vi "Read ApplicationRef.vi"(8 "error in (no error)":errorcluster, 11 "Test Runner in":refnum<class "Test Runner.lvclass">) -> (0 "error out":errorcluster, 2 "Application":refnum<vi>, 3 "Test Runner out":refnum<class "Test Runner.lvclass">)   [LabVIEW 2020, in "Caraya.lvlib" / "Test Runner.lvclass"]
uses:
  Test Runner.lvclass
  Test Runner.lvclass/Test Runner.ctl
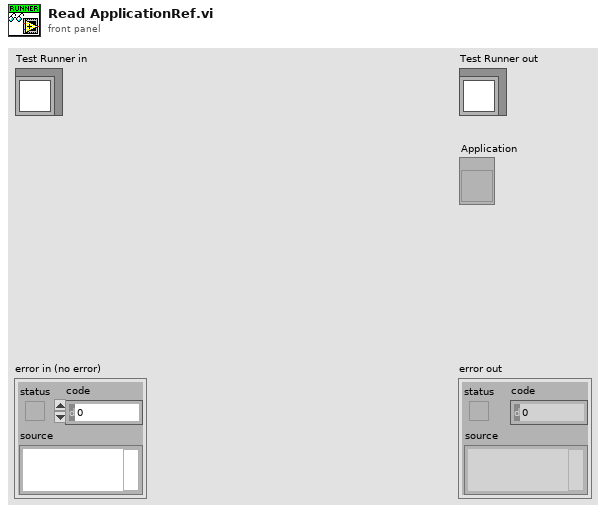
[diagram p1: front panel]
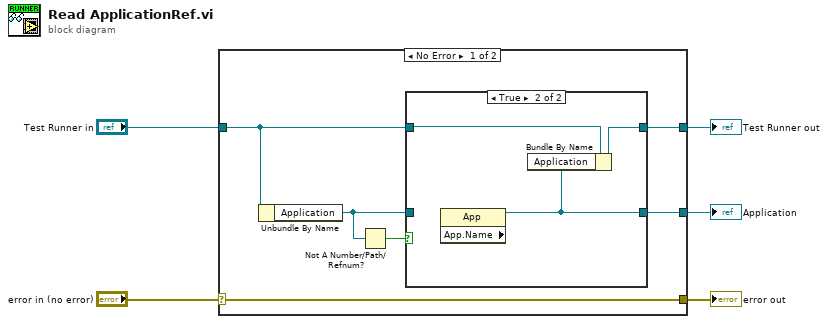
[diagram p0: block diagram]
diagram:
  n1 = case shown="No Error" "error in (no error)" {
    selector: "error in (no error)" -> [w11 w17]
    tunnel: [w11 w17] -> w4
    tunnel: [w7 w18] -> w2
    tunnel: "Test Runner in" -> [w6 w18]
    tunnel: [w8 _] -> w1
    frame No Error {
      n2 = Unbundle By Name(w6) -> ("Application"=w9:refnum<vi>)
      n3 = Not A Number/Path/Refnum?(number/path/refnum=w9) -> (NaN/Path/Refnum?=w10:bool)
      n4 = case shown="True" w10 {
        tunnel: w9 -> [w13 _]
        tunnel: [w13 w14] -> w8
        tunnel: [w12 w15] -> w7
        tunnel: w6 -> [w12 w16]
        frame False {
        }
        frame True {
          n5 = property class="App" props=["App.Name"]() -> (reference out=w14:refnum<vi>)  [unwired: 2 in, 2 out]
          n6 = Bundle By Name(cluster=w16, "Application"=w14) -> (w15:refnum<class "Test Runner.lvclass">)
        }
      }
    }
    frame Error {
    }
  }
  "error out" <- w4
  "Test Runner out" <- w2
  "Application" <- w1
